vi "Initialize.vi"(8 "error in (no error)":errorcluster, 11 "ActivationHandler in":refnum<class "ActivationHandler.lvclass">) -> (0 "error out":errorcluster, 3 "ActivationHandler out":refnum<class "ActivationHandler.lvclass">)   [LabVIEW 2026, in "ToastNotification.lvlib" / "ActivationHandler.lvclass"]
doc: "Initialization hook for activation handlers. The base implementation passes the handler and error through without acquiring resources. Override in a child class to create resources needed by Handle Activation. ToastService.Initialize invokes this hook and stores the returned initialized handler. Define matching cleanup in Close."
uses:
  ActivationHandler.lvclass
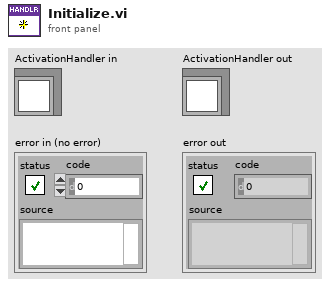
[diagram p1: front panel]
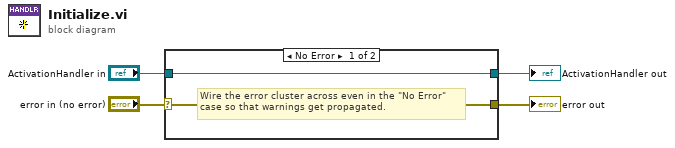
[diagram p0: block diagram]
diagram:
  n1 = case shown="No Error" "error in (no error)" {
    selector: "error in (no error)" -> [w5 w8]
    tunnel: [w5 w8] -> w3
    tunnel: [w6 w7] -> w1
    tunnel: "ActivationHandler in" -> [w6 w7]
    frame No Error {
      # "Wire the error cluster across even in the \"No Error\"\ncase so that warnings get propagated."
    }
    frame Error {
    }
  }
  "error out" <- w3
  "ActivationHandler out" <- w1
